vi "wiringPiVersion.vi"(8 "error in (no error)":errorcluster) -> (0 "error out":errorcluster, 2 "minor":i32, 3 "mayor":i32)   [LabVIEW 2020, in "wiringPi.lvlib"]
doc: "<b>_______________________________________________________________</b>\n** Author: Juan José Villacorta\n** LabVIEW wrapper for C library <b> wiringPi </b>,\n** https://github.com/WiringPi/WiringPi\n<b>_______________________________________________________________</b>\n\n\n/*\n * wiringPiVersion:\n * Return our current version number\n *********************************************************************************\n */"
uses:
  wiringPi.lvlib
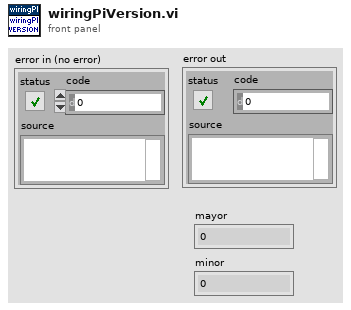
[diagram p1: front panel]
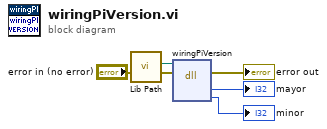
[diagram p0: block diagram]
diagram:
  n1 = call "Lib Path.vi"() -> ("path out"=w1:path)  [unwired: 11 in]
  n2 = dll-call lib="libLV_wiringPi.so" fn="wiringPiVersion"(path in=w1, error in="error in (no error)") -> (error out=→"error out":errorcluster, "major"=→"mayor":i32, "minor"=→"minor":i32)  [unwired: 4 in, 1 out]
